vi "Create Message Data Clusters (complex).vi"(8 "error in (no error)":errorcluster, 9 "generate serialization helpers":bool, 10 "message metadata":T1, 11 "library in":refnum<vi>) -> (0 "error out":errorcluster, 3 "library out":refnum<vi>)   [LabVIEW 2019, in "gRPC Template Creation Utility.lvlib"]
uses:
  gRPC Template Creation Utility.lvlib
  TypeDefs/Message Metadata (Scripting).ctl
  TypeDefs/Message Element Metadata (Scripting).ctl
  TypeDefs/Message Element Type.ctl
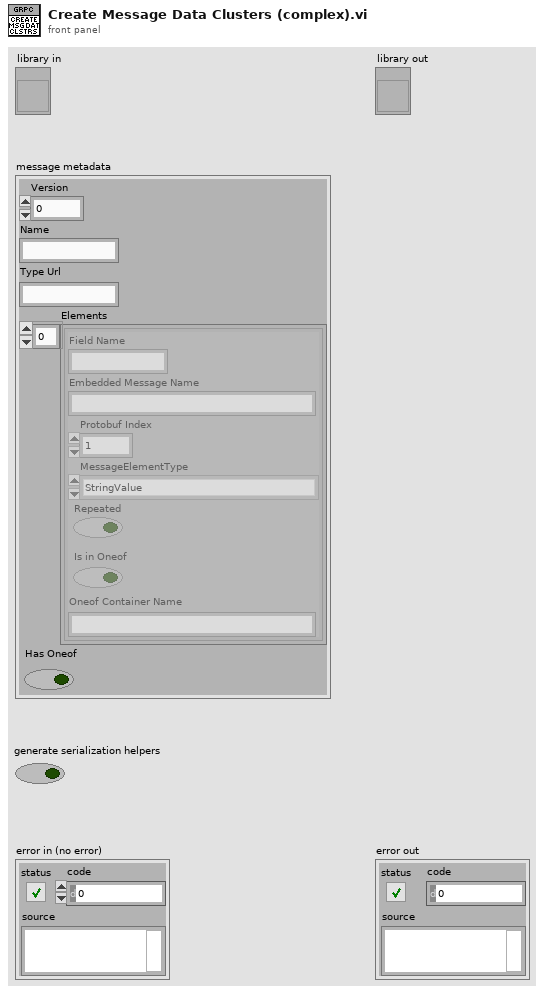
[diagram p1: front panel]
types:
  T1 = typedef "gRPC Template Creation Utility.lvlib/Message Metadata (Scripting).ctl" = cluster{"Version":i32, "Name":string, "Type Url":string, "Elements":T2[], "Has Oneof":bool}
  T2 = typedef "gRPC Template Creation Utility.lvlib/Message Element Metadata (Scripting).ctl" = cluster{"Field Name":string, "Embedded Message Name":string, "Protobuf Index":i32, "MessageElementType":T3, "Repeated":bool, "Is in Oneof":bool, "Oneof Container Name":string}
  T3 = typedef "gRPC Template Creation Utility.lvlib/Message Element Type.ctl" = enum32{"Int32Value", "FloatValue", "DoubleValue", "BoolValue", "StringValue", "MessageValue", "Int64Value", "UInt32Value", "UInt64Value", "EnumValue", "Bytes", "Fixed64", "Fixed32", "SFixed64", "SFixed32", "SInt64", "SInt32"}
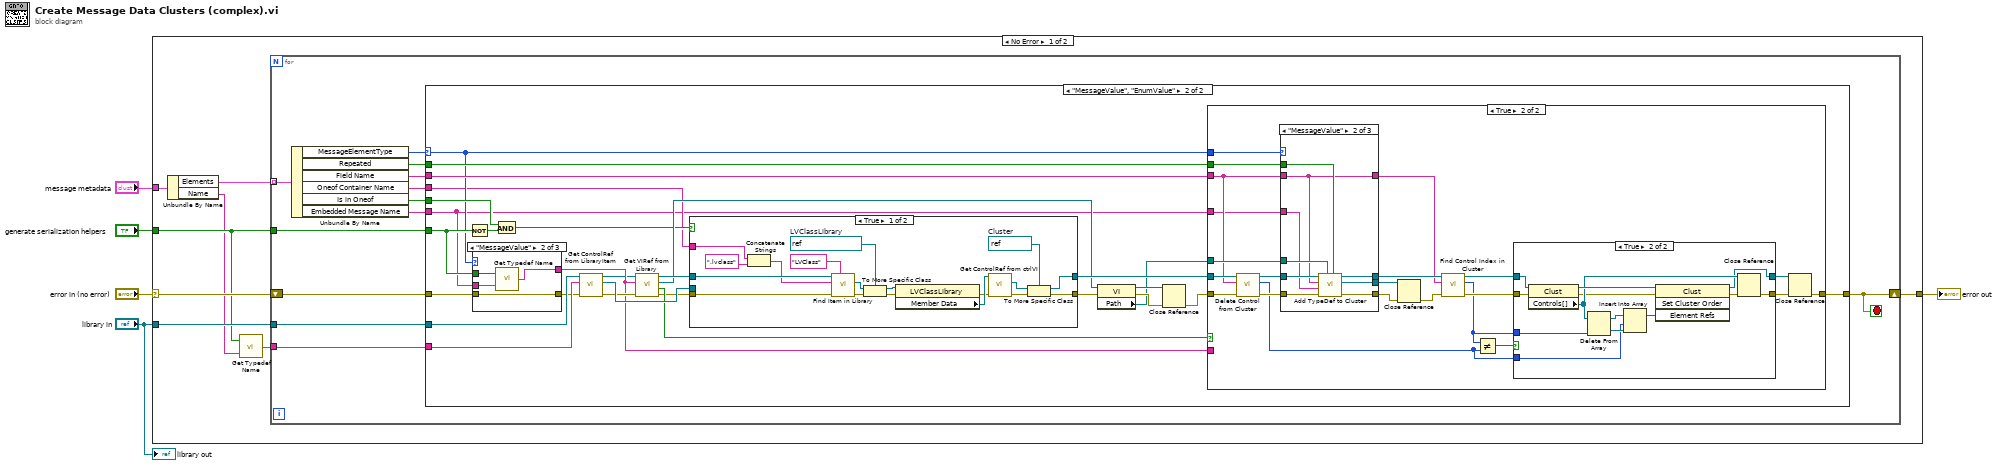
[diagram p0: block diagram]
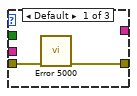
[diagram p3: hidden frame]
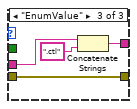
[diagram p4: hidden frame]
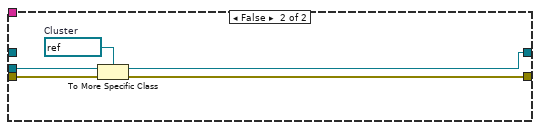
[diagram p5: hidden frame]
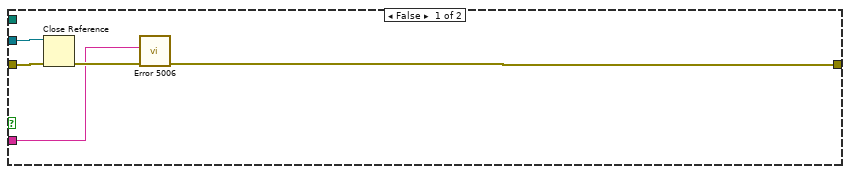
[diagram p6: hidden frame]
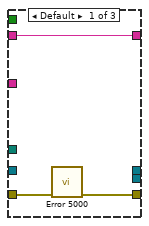
[diagram p7: hidden frame]
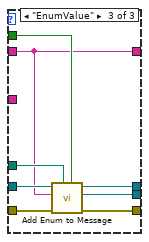
[diagram p8: hidden frame]
diagram:
  n1 = case shown="No Error" "error in (no error)" {
    selector: "error in (no error)" -> [w9 w150]
    tunnel: "message metadata" -> [w13 _]
    tunnel: "library in" -> [w10 _]
    tunnel: [w11 w150] -> w4
    tunnel: "generate serialization helpers" -> [w7 _]
    frame No Error {
      n2 = Unbundle By Name(w13) -> ("Elements"=w12:T2[], "Name"=w6:string)
      n3 = call "Get Typedef Name.vi"("embedded message name"=w6, "generate serialization helpers"=w7) -> ("typedef name"=w8:string)
      n4 = for {
        tunnel: w12 -> [w24] mode=indexing
        shift-right: [w21] -> w11
        shift-left: w9 -> [w22]
        tunnel: w8 -> [w23]
        tunnel: w7 -> [w20]
        tunnel: w10 -> [w25]
        stop <- w21 stop-if-true
        n5 = Unbundle By Name(w24) -> ("MessageElementType"=w16:T3, "Repeated"=w19:bool, "Field Name"=w18:string, "Oneof Container Name"=w17:string, "Is in Oneof"=w14:bool, "Embedded Message Name"=w15:string)
        n6 = case shown="\"MessageValue\", \"EnumValue\"" w16 {
          selector: w16 -> [_ w29]
          tunnel: w25 -> [_ w54]
          tunnel: w23 -> [_ w51]
          tunnel: w22 -> [w26 w31]
          tunnel: [w26 w37] -> w21
          tunnel: w20 -> [_ w44]
          tunnel: w19 -> [_ w34]
          tunnel: w18 -> [_ w33]
          tunnel: w14 -> [_ w32]
          tunnel: w17 -> [_ w28]
          tunnel: w15 -> [_ w27]
          frame Default {
          }
          frame "MessageValue", "EnumValue" {
            n7 = Not(x=w44) -> (.not. x?=w43:bool)
            n8 = case shown="\"MessageValue\"" w29 {
              tunnel: [_ w60 w62] -> w50
              tunnel: w44 -> [_ w59 _]
              tunnel: w27 -> [_ w58 w63]
              tunnel: w31 -> [w56 w57 w61]
              tunnel: [w55 w57 w61] -> w30
              frame Default {
                n9 = call "Error 5000.vi"("error in (no error)"=w56) -> ("error out"=w55:errorcluster)  [unwired: 10 in]
              }
              frame "MessageValue" {
                n10 = call "Get Typedef Name.vi"("embedded message name"=w58, "generate serialization helpers"=w59) -> ("typedef name"=w60:string)
              }
              frame "EnumValue" {
                n11 = Concatenate Strings(w63, ".ctl" ("string")) -> (w62:string)
              }
            }
            n12 = And(x=w32, y=w43) -> (x .and. y?=w35:bool)
            n13 = call "Get ControlRef from LibraryItem.vi"("error in (no error)"=w30, "Control Name"=w51, "Library item in"=w54) -> ("error out"=w52:errorcluster, "Control ref out"=w53:refnum<vi>, "Library item out"=w46:refnum<vi>)  [unwired: 5 in, 1 out]
            n14 = call "Get VIRef from Library.vi"("error in (no error)"=w52, "item name"=w50, "library in"=w46) -> ("error out"=w47:errorcluster, "found"=w48:bool, "vi"=w42:refnum<vi>, "library out"=w45:refnum<vi>)  [unwired: 5 in]
            n15 = case shown="True" w35 {
              tunnel: w53 -> [_ w87]
              tunnel: [w73 w85] -> w49
              tunnel: w47 -> [w80 w84]
              tunnel: [w66 w83] -> w38
              tunnel: w45 -> [w82 _]
              tunnel: w28 -> [w72 _]
              frame True {
                w74 = refnum<vi> refnum  # Cluster
                w79 = refnum<vi> refnum  # LVClassLibrary
                n16 = Concatenate Strings(w72, ".lvclass" ("string")) -> (w70:string)
                n17 = call "Find Item in Library.vi"("Item Type"="LVClass", "error in (no error)"=w80, "Item Name"=w70, "Library item in"=w82) -> ("error out"=w78:errorcluster, "Project Item (Library Item)"=w77:refnum<vi>)  [unwired: 4 in, 2 out]
                n18 = To More Specific Class(target class=w79, reference=w77, error in=w78) -> (specific class reference=w76:refnum<vi>, error out=w75:errorcluster)
                n19 = property class="LVClassLibrary"(reference=w76, error in=w75) -> (error out=w67:errorcluster, "Member Data"=w69:refnum<vi>)  [unwired: 1 out]
                n20 = call "Get ControlRef from ctrlVI.vi"("error in (no error)"=w67, "VI ref in"=w69) -> ("error out"=w65:errorcluster, "Control ref out"=w68:refnum<vi>)  [unwired: 7 in, 1 out]
                n21 = To More Specific Class(target class=w74, reference=w68, error in=w65) -> (specific class reference=w73:refnum<vi>, error out=w66:errorcluster)
              }
              frame False {
                w86 = refnum<vi> refnum  # Cluster
                n22 = To More Specific Class(target class=w86, reference=w87, error in=w84) -> (specific class reference=w85:refnum<vi>, error out=w83:errorcluster)
              }
            }
            n23 = property class="VI"(reference=w42, error in=w38) -> (reference out=w40:refnum<vi>, error out=w41:errorcluster, "Path"=w36:path)
            n24 = Close Reference(reference=w40, error in (no error)=w41) -> (error out=w39:errorcluster)
            n25 = case shown="True" w48 {
              tunnel: w49 -> [w92 w114]
              tunnel: [w89 w97] -> w37
              tunnel: w39 -> [w91 w107]
              tunnel: w33 -> [_ w95]
              tunnel: w34 -> [_ w99]
              tunnel: w50 -> [w88 _]
              tunnel: w36 -> [_ w98]
              tunnel: w29 -> [_ w96]
              tunnel: w27 -> [_ w93]
              frame False {
                n26 = Close Reference(reference=w92, error in (no error)=w91) -> (error out=w90:errorcluster)
                n27 = call "Error 5006.vi"("error in (no error)"=w90, "Embedded Message Name"=w88) -> ("error out"=w89:errorcluster)  [unwired: 9 in]
              }
              frame True {
                n28 = call "Delete Control from Cluster.vi"("error in (no error)"=w107, "Control Name in"=w95, "Cluster ref in"=w114) -> ("error out"=w106:errorcluster, "Deleted Index"=w100:i32, "Cluster ref out"=w105:refnum<vi>)  [unwired: 6 in]
                n29 = case shown="\"MessageValue\"" w96 {
                  tunnel: w106 -> [w117 w126 w134]
                  tunnel: w105 -> [_ w125 w130]
                  tunnel: [_ w124 w132] -> w104
                  tunnel: [_ w123 w131] -> w103
                  tunnel: [w116 w122 w133] -> w102
                  tunnel: w99 -> [_ w121 w129]
                  tunnel: w98 -> [_ w120 w128]
                  tunnel: w95 -> [w115 w119 w127]
                  tunnel: [w115 w119 w127] -> w94
                  tunnel: w93 -> [_ w118 _]
                  frame Default {
                    n30 = call "Error 5000.vi"("error in (no error)"=w117) -> ("error out"=w116:errorcluster)  [unwired: 10 in]
                  }
                  frame "MessageValue" {
                    n31 = call "Add TypeDef to Cluster.vi"("isArray (F)"=w121, "TypeDef path"=w120, "error in (no error)"=w126, "field message name"=w118, "Field Name"=w119, "Owning cluster ref in"=w125) -> ("error out"=w122:errorcluster, "Control ref out"=w123:refnum<vi>, "Owning cluster ref out"=w124:refnum<vi>)  [unwired: 3 in]
                  }
                  frame "EnumValue" {
                    n32 = call "Add Enum to Message.vi"("isArray (F)"=w129, "TypeDef path"=w128, "error in (no error)"=w134, "Field Name"=w127, "Owning cluster ref in"=w130) -> ("error out"=w133:errorcluster, "Control ref out"=w131:refnum<vi>, "Owning cluster ref out"=w132:refnum<vi>)  [unwired: 4 in]
                  }
                }
                n33 = Close Reference(reference=w103, error in (no error)=w102) -> (error out=w101:errorcluster)
                n34 = call "Find Control Index in Cluster.vi"("error in (no error)"=w101, "Control Name"=w94, "Cluster ref in"=w104) -> ("error out"=w111:errorcluster, "Control Index"=w110:i32, "Cluster ref out"=w112:refnum<vi>)  [unwired: 6 in]
                n35 = Not Equal?(x=w110, y=w100) -> (x != y?=w113:bool)
                n36 = case shown="True" w113 {
                  tunnel: w112 -> [w135 w149]
                  tunnel: w111 -> [w136 w148]
                  tunnel: w110 -> [_ w147]
                  tunnel: w100 -> [_ w144]
                  tunnel: [w136 w139] -> w109
                  tunnel: [w135 w138] -> w108
                  frame False {
                  }
                  frame True {
                    n37 = property class="Clust"(reference=w149, error in=w148) -> (reference out=w143:refnum<vi>, error out=w137:errorcluster, "Controls[]"=w140:refnum<vi>[])
                    n38 = Delete From Array(array=w140, index=w147) -> (deleted portion=w145:refnum<vi>, array with subset deleted=w146:refnum<vi>[])  [unwired: 1 in]
                    n39 = Insert Into Array(array=w146, index=w144, new element=w145) -> (w142:refnum<vi>[])
                    n40 = invoke class="Clust" method="Set Cluster Order"(reference=w143, error in=w137, "Element Refs"=w142) -> (reference out=w138:refnum<vi>, error out=w141:errorcluster)  [unwired: 1 in, 2 out]
                    n41 = Close Reference(reference=w140, error in (no error)=w141) -> (error out=w139:errorcluster)
                  }
                }
                n42 = Close Reference(reference=w108, error in (no error)=w109) -> (error out=w97:errorcluster)
              }
            }
          }
        }
      }
    }
    frame Error {
    }
  }
  "error out" <- w4
  "library out" <- "library in"
